vi "RDC-water-read_parameter.vi"() -> (2 "water param Array":T1[](array[typedef]), 3 "water param map":map{u16, T1}(c390))   [LabVIEW 2020, in "RDC-Reflection_Data_Computation.lvlib"]
doc: "Parses the water parameter table stored in the VI (T, e_s, e_inf, tau and their uncertainties) into an array and a map keyed by temperature x10."
uses:
  RDC-Reflection_Data_Computation.lvlib
  RDC-water-param.ctl
panel:
  out "string array":string[](array[string])
  out "array w/ subset deleted":string[](array[string])
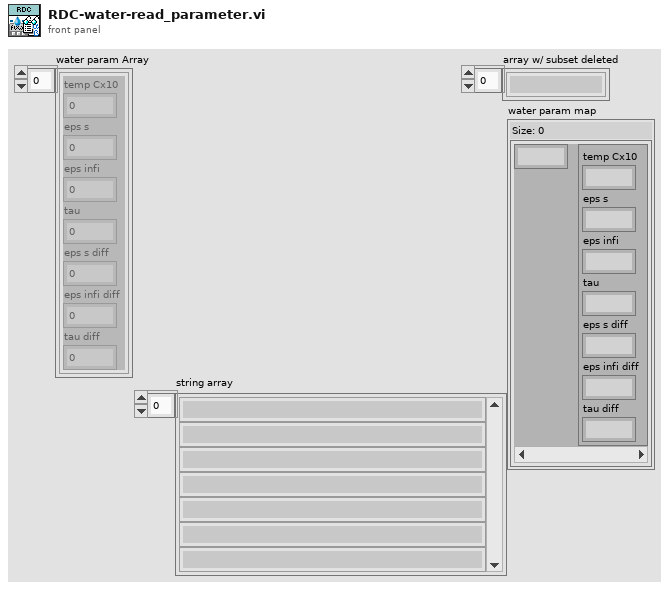
[diagram p1: front panel]
types:
  T1 = typedef "RDC-Reflection_Data_Computation.lvlib/RDC-water-param.ctl" = cluster{"temp Cx10":u16, "eps s":dbl, "eps infi":dbl, "tau":dbl, "eps s diff":dbl, "eps infi diff":dbl, "tau diff":dbl}
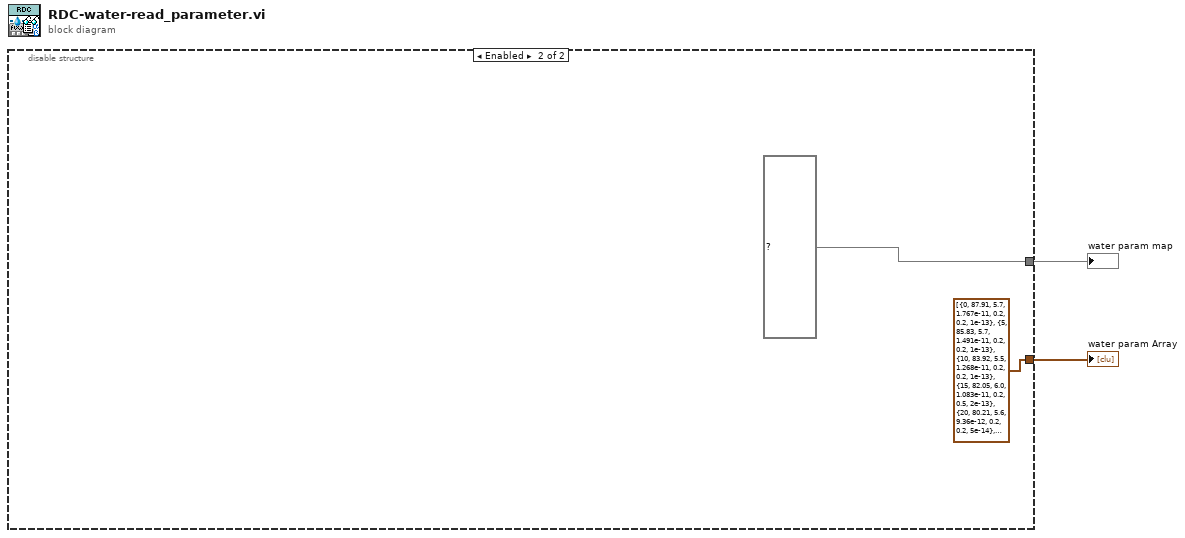
[diagram p0: block diagram]
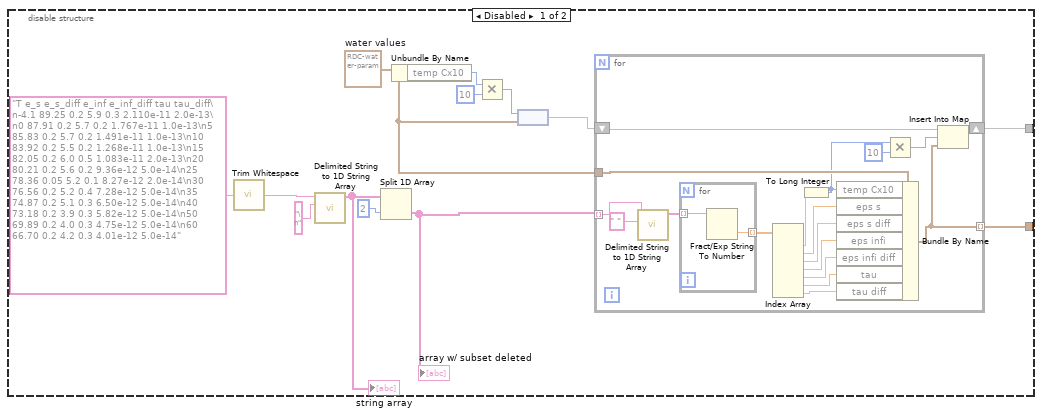
[diagram p2: hidden frame]
diagram:
  n1 = disable-structure shown="Enabled" {
    disable-tunnel: [w5 map{u16, T1} {} ("water param map 2")] -> w2
    disable-tunnel: [w4 T1[] [{"temp Cx10"=0, "eps s"=87.91, "eps infi"=5.7, "tau"=1.767e-11, "eps s diff"=0.2, "eps infi diff"=0.2, "tau diff"=1e-13}, {"temp Cx10"=5, "eps s"=85.83, "eps infi"=5.7, "tau"=1.491e-11, "eps s diff"=0.2, "eps infi diff"=0.2, "tau diff"=1e-13}, {"temp Cx10"=10, "eps s"=83.92, "eps infi"=5.5, "tau"=1.268e-11, "eps s diff"=0.2, "eps infi diff"=0.2, "tau diff"=1e-13}, {"temp Cx10"=15, "eps s"=82.05, "eps infi"=6.0, "tau"=1.083e-11, "eps s diff"=0.2, "eps infi diff"=0.5, "tau diff"=2e-13}, {"temp Cx10"=20, "eps s"=80.21, "eps infi"=5.6, "tau"=9.36e-12, "eps s diff"=0.2, "eps infi diff"=0.2, "tau diff"=5e-14}, {"temp Cx10"=25, "eps s"=78.36, "eps infi"=5.2, "tau"=8.27e-12, "eps s diff"=0.05, "eps infi diff"=0.1, "tau diff"=2e-14}, {"temp Cx10"=30, "eps s"=76.56, "eps infi"=5.2, "tau"=7.28e-12, "eps s diff"=0.2, "eps infi diff"=0.4, "tau diff"=5e-14}, {"temp Cx10"=35, "eps s"=74.87, "eps infi"=5.1, "tau"=6.5e-12, "eps s diff"=0.2, "eps infi diff"=0.3, "tau diff"=5e-14}, {"temp Cx10"=40, "eps s"=73.18, "eps infi"=3.9, "tau"=5.82e-12, "eps s diff"=0.2, "eps infi diff"=0.3, "tau diff"=5e-14}, {"temp Cx10"=50, "eps s"=69.89, "eps infi"=4.0, "tau"=4.75e-12, "eps s diff"=0.2, "eps infi diff"=0.3, "tau diff"=5e-14}, {"temp Cx10"=60, "eps s"=66.7, "eps infi"=4.2, "tau"=4.01e-12, "eps s diff"=0.2, "eps infi diff"=0.3, "tau diff"=5e-14}] ("water param Array 2")] -> w1
    frame Disabled {
      w6 = T1 {"temp Cx10"=25, "eps s"=78.36, "eps infi"=5.2, "tau"=8.27e-12, "eps s diff"=78.36, "eps infi diff"=5.2, "tau diff"=8.27e-12}  # water values
      n2 = call <vilib>:"Trim Whitespace.vi"("string"="T e_s e_s_diff e_inf e_inf_diff tau tau_diff\n-4.1 89.25 0.2 5.9 0.3 2.110e-11 2.0e-13\n0 87.91 0.2 5.7 0.2 1.767e-11 1.0e-13\n5 85.83 0.2 5.7 0.2 1.491e-11 1.0e-13\n10 83.92 0.2 5.5 0.2 1.268e-11 1.0e-13\n15 82.05 0.2 6.0 0.5 1.083e-11 2.0e-13\n20 80.21 0.2 5.6 0.2 9.36e-12 5.0e-14\n25 78.36 0.05 5.2 0.1 8.27e-12 2.0e-14\n30 76.56 0.2 5.2 0.4 7.28e-12 5.0e-14\n35 74.87 0.2 5.1 0.3 6.50e-12 5.0e-14\n40 73.18 0.2 3.9 0.3 5.82e-12 5.0e-14\n50 69.89 0.2 4.0 0.3 4.75e-12 5.0e-14\n60 66.70 0.2 4.2 0.3 4.01e-12 5.0e-14") -> ("trimmed string"=w3:string)  [unwired: 1 in]
      n3 = call <vilib>:"Delimited String to 1D String Array.vi"("delimiter"="\n", "delimited string"=w3) -> ("string array"=w13:string[])  [unwired: 9 in]
      "string array" <- w13
      n4 = Split 1D Array(array=w13, index=2) -> (second subarray=w12:string[])  [unwired: 1 out]
      "array w/ subset deleted" <- w12
      n5 = Unbundle By Name(w6) -> ("temp Cx10"=w10:u16)
      n6 = Multiply(x=w10, y=u16 10) -> (x*y=w7:u16)
      n7 = node(w7, w6) -> (w8:map{u16, T1})
      n8 = for {
        tunnel: w12 -> [w33] mode=indexing
        tunnel: w6 -> [w29]
        tunnel: [w16] -> w4 mode=indexing
        shift-right: [w20] -> w5
        shift-left: w8 -> [w21]
        n9 = call <vilib>:"Delimited String to 1D String Array.vi"("delimiter"=" ", "delimited string"=w33) -> ("string array"=w31:string[])  [unwired: 9 in]
        n10 = for {
          tunnel: w31 -> [w35] mode=indexing
          tunnel: [w34] -> w30 mode=indexing
          n11 = Fract/Exp String To Number(string=w35) -> (number=w34:dbl)  [unwired: 3 in, 1 out]
        }
        n12 = Index Array(array=w30) -> (element #1=w28:dbl, element #2=w27:dbl, element #3=w26:dbl, element #4=w25:dbl, element #5=w24:dbl, element #6=w23:dbl, element #7=w22:dbl)  [unwired: 7 in]
        n13 = To Long Integer(number=w28) -> (32bit integer=w18:i32)
        n14 = Bundle By Name(cluster=w29, "temp Cx10"=w18, "eps s"=w27, "eps s diff"=w26, "eps infi"=w25, "eps infi diff"=w24, "tau"=w23, "tau diff"=w22) -> (w16:T1)
        n15 = Multiply(x=w18, y=u16 10) -> (x*y=w17:i32)
        n16 = Insert Into Map(map in=w21, key=w17, value=w16) -> (map out=w20:map{u16, T1})  [unwired: 2 out]
      }
    }
    frame Enabled {
    }
  }
  "water param map" <- w2
  "water param Array" <- w1
